vi "Panel.vi"(7 "Set(F)":bool, 8 "error in (no error)":errorcluster, 10 "First Time(F)":bool, 11 "object in":refnum<class>) -> (0 "error out":errorcluster, 2 "Changed?":bool, 3 "object out":refnum<class>)   [LabVIEW 2021, in "Channel.lvlib" / "Configuration.lvclass"]
uses:
  Configuration.lvclass
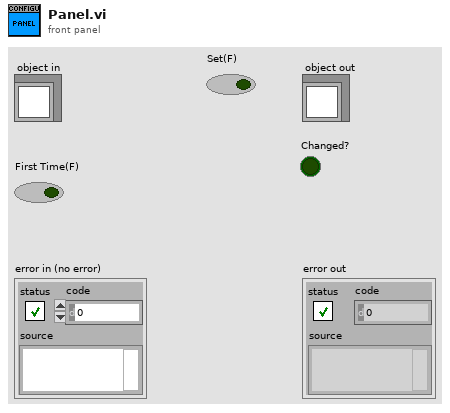
[diagram p1: front panel]
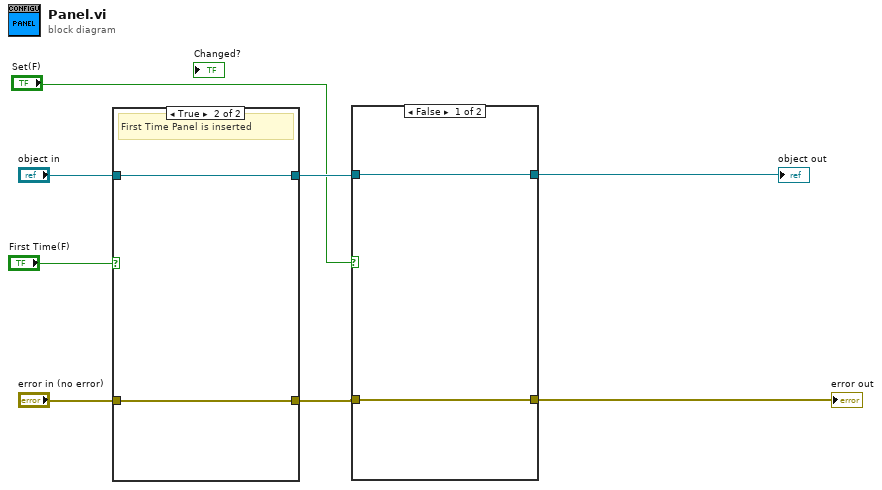
[diagram p0: block diagram]
diagram:
  n1 = case shown="True" "First Time(F)" {
    tunnel: [w10 w12] -> w5
    tunnel: "object in" -> [w10 w12]
    tunnel: [w9 w11] -> w3
    tunnel: "error in (no error)" -> [w9 w11]
    frame False {
    }
    frame True {
      # "First Time Panel is inserted"
    }
  }
  n2 = case shown="False" "Set(F)" {
    tunnel: [w14 w16] -> w4
    tunnel: w5 -> [w14 w16]
    tunnel: [w13 w15] -> w2
    tunnel: w3 -> [w13 w15]
    frame False {
    }
    frame True {
      # "Update controls with data in class"
    }
  }
  "error out" <- w2
  "object out" <- w4
